vi "MQTT Subscriptions - Handle Unsubscribe.vi"(0 "MQTT ref in":T1, 5 "Packet ID":u16, 7 "Topic Filters":string[](array[string]), 11 "error in":errorcluster) -> (4 "MQTT ref out":T1, 15 "error out":errorcluster)   [LabVIEW 2019, in "KoRE-MQTT.lvlib"]
doc: "Copyright (c) 2025 KoRElibs.com\nSPDX-License-Identifier: EUPL-1.2\n\nThis VI is licensed under the European Union Public License (EUPL) Version 1.2. You may use this VI unmodified in proprietary works. If you distribute a modified version of this file, the modified file must be released under the EUPL-1.2. Full license: https://joinup.ec.europa.eu/asset/eupl/eupl/1.2/"
uses:
  KoRE-MQTT.lvlib
  Public/TypeDefs/MQTT Client Session.ctl
  TypeDefs/MQTT Client Session - Data Value Reference.ctl
  Public/TypeDefs/MQTT Client Session - Data.ctl
  Public/TypeDefs/MQTT Property - Will.ctl
  Public/TypeDefs/MQTT Property - CONNECT.ctl
  TypeDefs/MQTT Subscription - Info.ctl
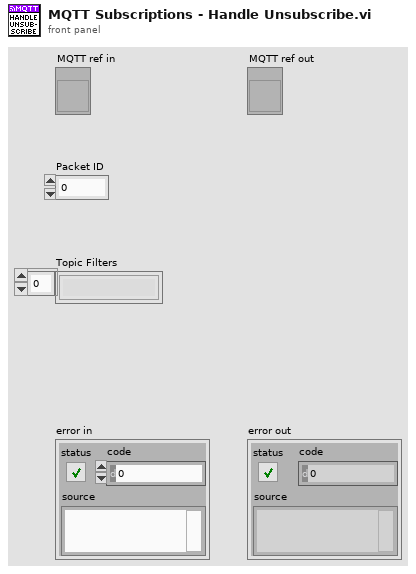
[diagram p1: front panel]
types:
  T1 = typedef "KoRE-MQTT.lvlib/MQTT Client Session.ctl" = refnum<vi>
  T2 = typedef "KoRE-MQTT.lvlib/MQTT Client Session - Data Value Reference.ctl" = refnum<data-value>
  T3 = typedef "KoRE-MQTT.lvlib/MQTT Subscription - Info.ctl" = cluster{"Packet Id":u16, "Index":u16, "Identifier":u32, "QoS":u8, "Topic Filter":string, "Reason Code":u8, "Reason String":string, "Granted":bool}
  T4 = typedef "KoRE-MQTT.lvlib/MQTT Client Session - Data.ctl" = cluster{"TCP ref":refnum<k5>, "Next Packet Id":u16, "Version":u8, "Host":string, "Port":u16, "Ping Delta":u32, "Username":string, "Password":string, "Will QoS":u8, "Will Retain":bool, "Will Topic":string, "Will Payload":string, "TCP Timeout":i32, "Semaphore":T5, "In-Flight Messages":variant, "Close":bool, "Last Send":u32, "Keep Alive":u16, "Last Ping RTT":u32, "Last Ping":u32, "Will Properties":T6[], "Session Expiry Interval":u32, "Maximum QoS":u8, "Retain Available":bool, "Server Maximum Packet Size":u32, "Client Identifier":string, "Server Topic Alias Maximum":u16, "Wildcard Subscription Available":bool, "Subscription Identifier Available":bool, "Shared Subscription Available":bool, "Connect Properties":T7[], "Client Maximum Packet Size":u32, "Client Topic Alias Maximum":u16, "Server Receive Maximum":u16, "Client Receive Maximum":u16, "TLS cfg":refnum<k36>, "Subscriptions":T3[]}
  T5 = typedef "Semaphore RefNum" = refnum<k1>
  T6 = typedef "KoRE-MQTT.lvlib/MQTT Property - Will.ctl" = cluster{"Property":u8, "Value":string}
  T7 = typedef "KoRE-MQTT.lvlib/MQTT Property - CONNECT.ctl" = cluster{"Property":u8, "Value":string}
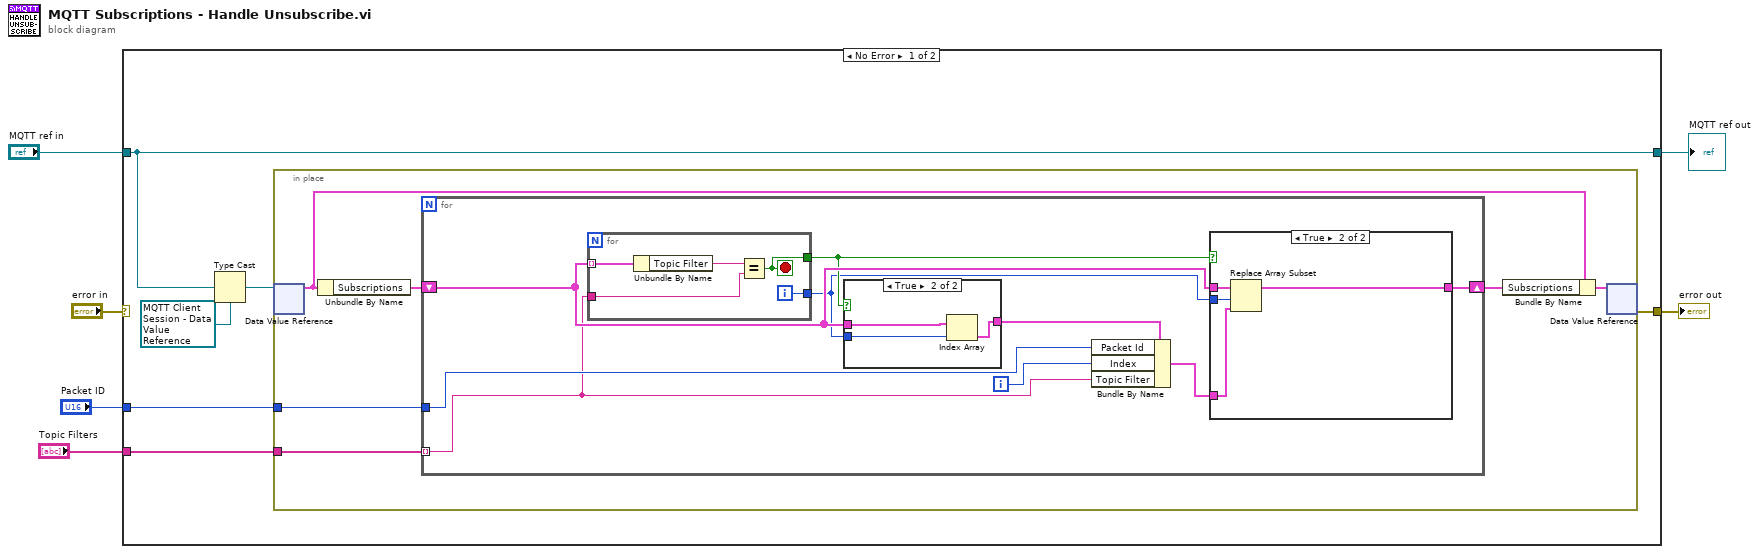
[diagram p0: block diagram]
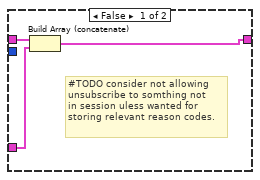
[diagram p2: hidden frame]
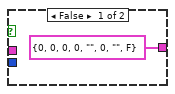
[diagram p3: hidden frame]
diagram:
  n1 = case shown="No Error" "error in" {
    selector: "error in" -> [_ w45]
    tunnel: "Packet ID" -> [w12 _]
    tunnel: "MQTT ref in" -> [w7 w44]
    tunnel: "Topic Filters" -> [w9 _]
    tunnel: [w8 w45] -> w3
    tunnel: [w7 w44] -> w1
    frame No Error {
      n2 = Type Cast(type=T2 refnum ("data value reference"), x=w7) -> (*(type *) &x=w11:T2)
      n3 = in-place {
        in-place-border: w12 -> [w18]
        in-place-border: w9 -> [w13]
        n4 = in-place-dvr #1(w11) -> (w14:T4)  [unwired: 1 out]
        n5 = Unbundle By Name(w14) -> ("Subscriptions"=w17:T3[])
        n6 = for {
          tunnel: w18 -> [w27]
          shift-right: [w22] -> w16
          shift-left: w17 -> [w24]
          tunnel: w13 -> [w19] mode=indexing
          i -> [w26]
          n7 = for {
            tunnel: w24 -> [w43] mode=indexing
            tunnel: w19 -> [w41]
            tunnel: [w40] -> w21
            tunnel: [w39] -> w20
            i -> [w39]
            stop <- w40 stop-if-true
            n8 = Unbundle By Name(w43) -> ("Topic Filter"=w42:string)
            n9 = Equal?(x=w42, y=w41) -> (x = y?=w40:bool)
          }
          n10 = case shown="True" w21 {
            tunnel: [T3 {"Packet Id"=0, "Index"=0, "Identifier"=0, "QoS"=0, "Topic Filter"="", "Reason Code"=0, "Reason String"="", "Granted"=FALSE} ("Subscription Info") w36] -> w25
            tunnel: w24 -> [_ w38]
            tunnel: w20 -> [_ w37]
            frame False {
            }
            frame True {
              n11 = Index Array(array=w38, index=w37) -> (element=w36:T3)
            }
          }
          n12 = Bundle By Name(cluster=w25, "Packet Id"=w27, "Index"=w26, "Topic Filter"=w19) -> (w23:T3)
          n13 = case shown="True" w21 {
            tunnel: w24 -> [w30 w34]
            tunnel: w23 -> [w29 w32]
            tunnel: [w28 w31] -> w22
            tunnel: w20 -> [_ w33]
            frame False {
              # "#TODO consider not allowing\nunsubscribe to somthing not\nin session uless wanted for\nstoring relevant reason codes."
              n14 = Build Array (concatenate)(w30, w29) -> (w28:T3[])
            }
            frame True {
              n15 = Replace Array Subset(array=w34, new element=w32, index=w33) -> (w31:T3[])
            }
          }
        }
        n16 = Bundle By Name(cluster=w14, "Subscriptions"=w16) -> (w15:T4)
        n17 = in-place-dvr #1(w15) -> (w8:errorcluster)  [unwired: 1 out]
      }
    }
    frame Error {
    }
  }
  "error out" <- w3
  "MQTT ref out" <- w1
